vi "ZM-launcher_test.vi"(9 "use_placeholder_hardware":bool, 10 "output_folder":path, 11 "run_time_ms":u32=5000) -> (0 "error out":errorcluster, 1 "error_lines":i32, 2 "last_line":string, 3 "lines_written":i32, 4 "ui_errors":string)   [LabVIEW 2020]
doc: "Headless test launcher of the actor tree. Deletes TestPackage.jsonl and the error log, launches the root with the given settings (placeholder hardware optional), waits run_time_ms, reads the root panel's errors, sends Normal Stop and counts the lines of both files. error out merges the launch, the panel read and the stop."
uses:
  actors/ZM-ROOT-root/ZM-ROOT-root/ZM-ROOT-root.lvclass
  <vilib>/ActorFramework/Stop Msg/Stop Msg.lvclass
  <vilib>/ActorFramework/Actor/Actor.lvclass
  actors/ZM-ROOT-root/ZM-ROOT-root/ZM-ROOT-PRELAUNCH_SETTINGS.ctl
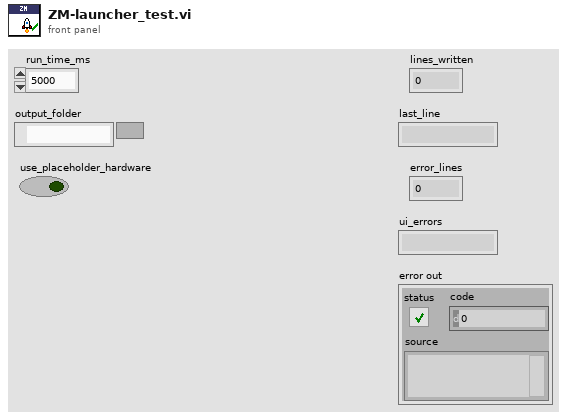
[diagram p1: front panel]
types:
  T1 = typedef "ZM-ROOT-root.lvlib/ZM-ROOT-root.lvclass/ZM-ROOT-PRELAUNCH_SETTINGS.ctl" = cluster{"outputFolder":path, "usePlaceholderHardware":bool}
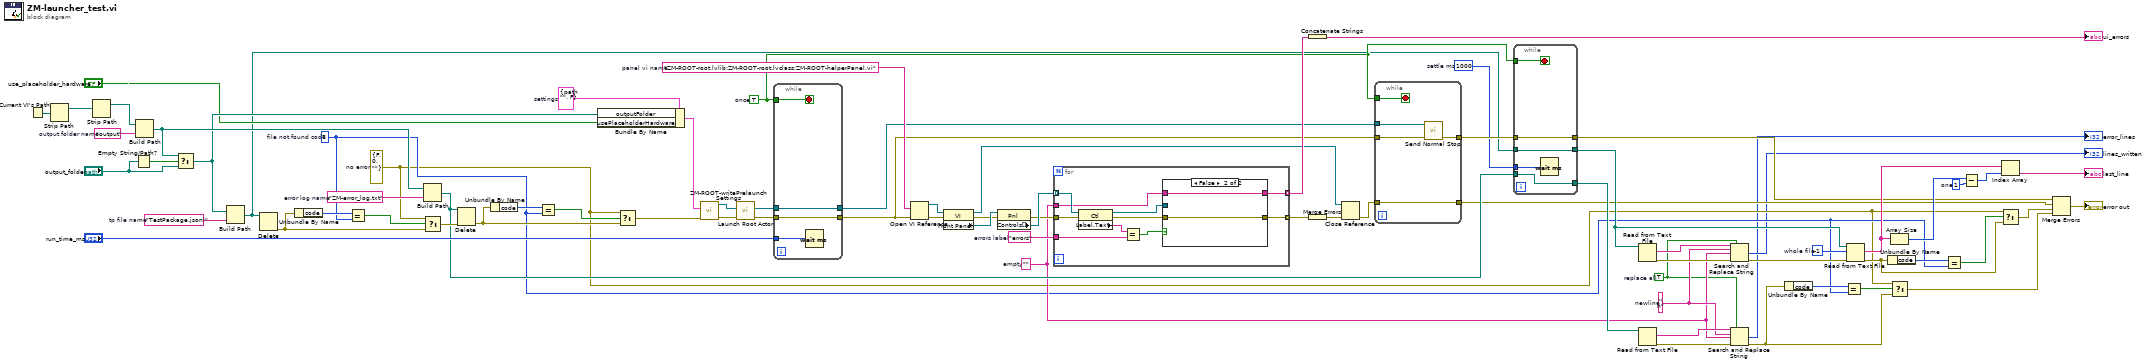
[diagram p0: block diagram]
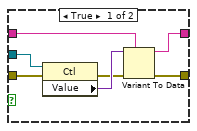
[diagram p2: hidden frame]
diagram:
  w26 = 1  # one
  w29 = -1  # whole file
  w46 = "errors"  # errors label
  w52 = "ZM-ROOT-root.lvlib:ZM-ROOT-root.lvclass:ZM-ROOT-helperPanel.vi"  # panel vi name
  w35 = u32 1000  # settle ms
  w36 = TRUE  # once
  w15 = TRUE  # replace all
  w17 = ""  # empty
  w18 = "\n"  # newline
  w12 = errorcluster {"status"=FALSE, "code"=0, "source"=""}  # no error
  w13 = 7  # file not found code
  w70 = "ZM-error_log.txt"  # error log name
  w72 = "TestPackage.jsonl"  # tp file name
  w75 = "output"  # output folder name
  w60 = T1 {"outputFolder"=path "", "usePlaceholderHardware"=FALSE}  # settings
  n1 = Current VI's Path() -> (path=w78:path)
  n2 = Strip Path(path=w78) -> (stripped path=w77:path)  [unwired: 1 out]
  n3 = Strip Path(path=w77) -> (stripped path=w76:path)  [unwired: 1 out]
  n4 = Empty String/Path?(string/path="output_folder") -> (empty?=w74:bool)
  n5 = Build Path(base path=w76, name or relative path=w75) -> (appended path=w71:path)
  n6 = Select(t=w71, s=w74, f="output_folder") -> (s? t:f=w62:path)
  n7 = Build Path(base path=w62, name or relative path=w72) -> (appended path=w34:path)
  n8 = Delete(path (use dialog)=w34) -> (error out=w67:errorcluster)  [unwired: 4 in, 2 out]
  n9 = Unbundle By Name(w67) -> ("code"=w69:i32)
  n10 = Equal?(x=w69, y=w13) -> (x = y?=w68:bool)
  n11 = Build Path(base path=w71, name or relative path=w70) -> (appended path=w33:path)
  n12 = Select(t=w12, s=w68, f=w67) -> (s? t:f=w66:errorcluster)
  n13 = Delete(path (use dialog)=w33, error in=w66) -> (error out=w63:errorcluster)  [unwired: 3 in, 2 out]
  n14 = Unbundle By Name(w63) -> ("code"=w65:i32)
  n15 = Equal?(x=w65, y=w13) -> (x = y?=w64:bool)
  n16 = Bundle By Name(cluster=w60, "outputFolder"=w62, "usePlaceholderHardware"="use_placeholder_hardware") -> (w59:T1)
  n17 = Select(t=w12, s=w64, f=w63) -> (s? t:f=w58:errorcluster)
  n18 = call "ZM-ROOT-writePrelaunchSettings.vi"("error in (no error)"=w58, "settings"=w59) -> ("error out"=w56:errorcluster, "ZM-ROOT-root out"=w57:refnum<class "ZM-ROOT-root.lvclass">)  [unwired: 8 in]
  n19 = call <vilib>:"Launch Root Actor.vi"("error in (no error)"=w56, "Actor"=w57) -> ("error out"=w55:errorcluster, "Actor's Enqueuer"=w54:refnum<class "Message Enqueuer.lvclass">)  [unwired: 8 in]
  n20 = while {
    tunnel: w55 -> [w80]
    tunnel: w36 -> [w81]
    tunnel: w54 -> [w79]
    tunnel: "run_time_ms" -> [w82]
    tunnel: [w80] -> w40
    tunnel: [w79] -> w39
    stop <- w81 stop-if-true
    n21 = Wait (ms)(milliseconds to wait=w82) -> ()  [unwired: 1 out]
  }
  n22 = Open VI Reference(vi path=w52, error in (no error)=w40) -> (vi reference=w51:refnum<vi>, error out=w50:errorcluster)  [unwired: 4 in]
  n23 = property class="VI"(reference=w51, error in=w50) -> (reference out=w42:refnum<vi>, error out=w48:errorcluster, "Front Panel"=w49:refnum<vi>)
  n24 = property class="Pnl"(reference=w49, error in=w48) -> (error out=w45:errorcluster, "Controls[]"=w47:refnum<vi>[])  [unwired: 1 out]
  n25 = for {
    tunnel: w47 -> [w92] mode=indexing
    tunnel: w46 -> [w89]
    tunnel: w45 -> [w91]
    tunnel: w17 -> [w87]
    tunnel: [w84] -> w44 mode=indexing
    tunnel: [w83] -> w43 mode=indexing
    n26 = property class="Ctl"(reference=w92, error in=w91) -> (reference out=w88:refnum<vi>, error out=w86:errorcluster, "Label.Text"=w90:string)
    n27 = Equal?(x=w90, y=w89) -> (x = y?=w85:bool)
    n28 = case shown="False" w85 {
      tunnel: w88 -> [w99 _]
      tunnel: w87 -> [w96 w100]
      tunnel: w86 -> [w98 w101]
      tunnel: [w94 w101] -> w84
      tunnel: [w93 w100] -> w83
      frame True {
        n29 = property class="Ctl"(reference=w99, error in=w98) -> (error out=w95:errorcluster, "Value"=w97:variant)  [unwired: 1 out]
        n30 = Variant To Data(error in=w95, type=w96, Variant=w97) -> (data=w93:string, error out=w94:errorcluster)
      }
      frame False {
      }
    }
  }
  n31 = Concatenate Strings(w43) -> (→"ui_errors":string)
  n32 = Merge Errors(w44) -> (w41:errorcluster)
  n33 = Close Reference(reference=w42, error in (no error)=w41) -> (error out=w38:errorcluster)
  n34 = while {
    tunnel: w40 -> [w106]
    tunnel: w36 -> [w104]
    tunnel: w39 -> [w105]
    tunnel: w38 -> [w102]
    tunnel: [w103] -> w37
    tunnel: [w102] -> w8
    stop <- w104 stop-if-true
    n35 = call <vilib>:"Send Normal Stop.vi"("error in (no error)"=w106, "Message Enqueuer"=w105) -> ("error out"=w103:errorcluster)  [unwired: 9 in]
  }
  n36 = while {
    tunnel: w37 -> [w109]
    tunnel: w36 -> [w110]
    tunnel: w35 -> [w111]
    tunnel: w34 -> [w108]
    tunnel: w33 -> [w107]
    tunnel: [w109] -> w9
    tunnel: [w108] -> w30
    tunnel: [w107] -> w20
    stop <- w110 stop-if-true
    n37 = Wait (ms)(milliseconds to wait=w111) -> ()  [unwired: 1 out]
  }
  n38 = Read from Text File(file (use dialog)=w30) -> (text=w32:string, error out=w31:errorcluster)  [unwired: 3 in, 2 out]
  n39 = Read from Text File(file (use dialog)=w20) -> (text=w19:string, error out=w16:errorcluster)  [unwired: 3 in, 2 out]
  n40 = Search and Replace String(replace all?=w15, input string=w32, search string=w18, replace string=w17, error in=w31) -> (number of replacements=→"lines_written":i32, error out=w28:errorcluster)  [unwired: 3 in, 2 out]
  n41 = Search and Replace String(replace all?=w15, input string=w19, search string=w18, replace string=w17, error in=w16) -> (number of replacements=→"error_lines":i32, error out=w10:errorcluster)  [unwired: 3 in, 2 out]
  n42 = Unbundle By Name(w10) -> ("code"=w14:i32)
  n43 = Equal?(x=w14, y=w13) -> (x = y?=w11:bool)
  n44 = Read from Text File(file (use dialog)=w30, count=w29, error in=w28) -> (text=w25:string[], error out=w21:errorcluster)  [unwired: 1 in, 2 out]
  n45 = Unbundle By Name(w21) -> ("code"=w23:i32)
  n46 = Array Size(array=w25) -> (size(s)=w27:i32)
  n47 = Select(t=w12, s=w11, f=w10) -> (s? t:f=w6:errorcluster)
  n48 = Equal?(x=w23, y=w13) -> (x = y?=w22:bool)
  n49 = Subtract(x=w27, y=w26) -> (x-y=w24:i32)
  n50 = Index Array(array=w25, index=w24) -> (element=→"last_line":string)
  n51 = Select(t=w12, s=w22, f=w21) -> (s? t:f=w7:errorcluster)
  n52 = Merge Errors(w9, w8, w7, w6) -> (→"error out":errorcluster)
